vi "start_recovery_imaging__7a8101cc3c.vi"(8 "Pulses to start":u32, 9 "Total number of images to be acquired":i32=1000, 10 "interval between images (s)":dbl=0.01, 11 "Exposure (s)":dbl=0.0001) -> (3 "ReceivedCounts":u32)   [LabVIEW 2023]
doc: "This example demonstrates how to generate a finite number of digital pulses using a counter output.\n\nOn some hardware, this requires the use of a second counter to generate a gate signal. If necessary, DAQmx configures this second counter for you."
uses:
  <vilib>/DAQmx/miscellaneous.llb/DAQmx Fill In Error Info.vi
panel:
  out "task done?":bool
  out "array":cluster{dbl, dbl}[](array[cluster])
  in  "Stop 2":bool
  in  "Loop Time (ms)":u32=10
  # "Start Acquisition Settings"
  # "Camera Settings"
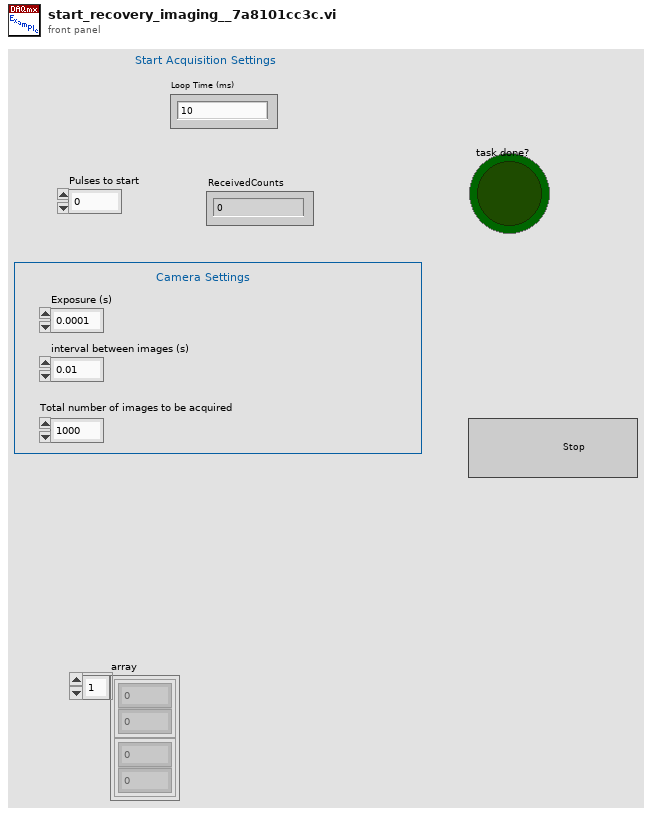
[diagram p1: front panel]
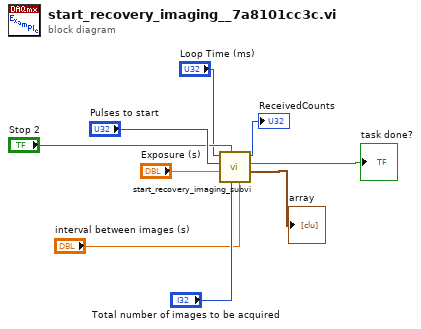
[diagram p0: block diagram]
diagram:
  n1 = call "start_recovery_imaging_subvi.vi"("interval between images (s)"="interval between images (s)", "Total number of images to be acquired"="Total number of images to be acquired", "Stop in"="Stop 2", "Exposure (s)"="Exposure (s)", "Pulses to start"="Pulses to start", "Loop Time (ms)"="Loop Time (ms)") -> ("array"=→"array":cluster{dbl, dbl}[], "task done?"=→"task done?":bool, "ReceivedCounts"=→"ReceivedCounts":u32)  [unwired: 3 in]
